vi "PicoScope5000aGetTriggerInfo.vi"(0 "handle in":i16, 5 "Rapid Block Acquisition Settings":T2 {"toSegmentIndex" format="%.4p"; "fromSegmentIndex" format="%.4p"}, 9 "Sample Rate":sgl, 11 "error in":errorcluster) -> (4 "handle out":i16, 6 "Trigger Info":T1(array[cluster]), 10 "Trigger Offsets":cluster{u64, sgl}[](array[cluster]) {"?" format="%#_5p"}, 15 "error out":errorcluster)   [LabVIEW 2010]
doc: "This VI gets a set of blocks captured using rapid block mode. It outputs two-dimensional arrays for each channel that contain data from all the requested captures."
uses:
  ps5000a.dll
  shared/Segment Range.ctl
panel:
  out "Number of Captures":u32=1
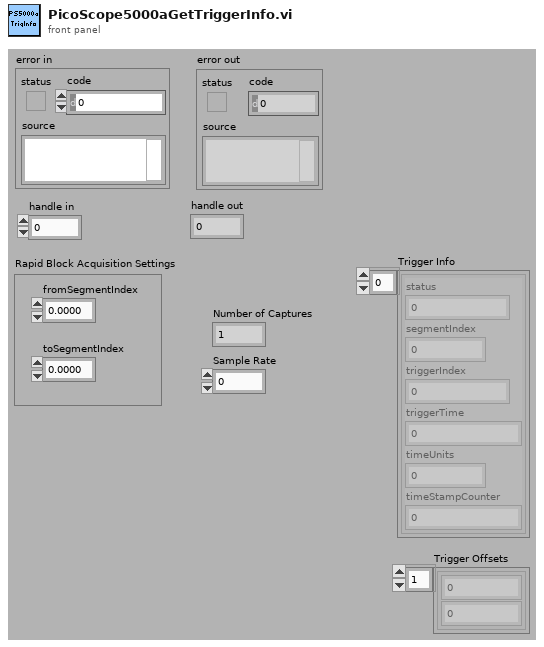
[diagram p1: front panel]
types:
  T1 = cluster{"status":u32, "segmentIndex":u32, "triggerIndex":u32, "triggerTime":i64, "timeUnits":i16, "timeStampCounter":u64}[]
  T2 = typedef "Segment Range.ctl" = cluster{"fromSegmentIndex":u64, "toSegmentIndex":u64}
  T3 = cluster{"status":u32, "segmentIndex":u32, "triggerIndex":u32, "triggerTime":i64, "timeUnits":i16, "reserved0":i16, "timeStampCounter":u64}
  T4 = cluster{"status":u32, "segmentIndex":u32, "triggerIndex":u32, "triggerTime":i64, "timeUnits":i16, "timeStampCounter":u64}
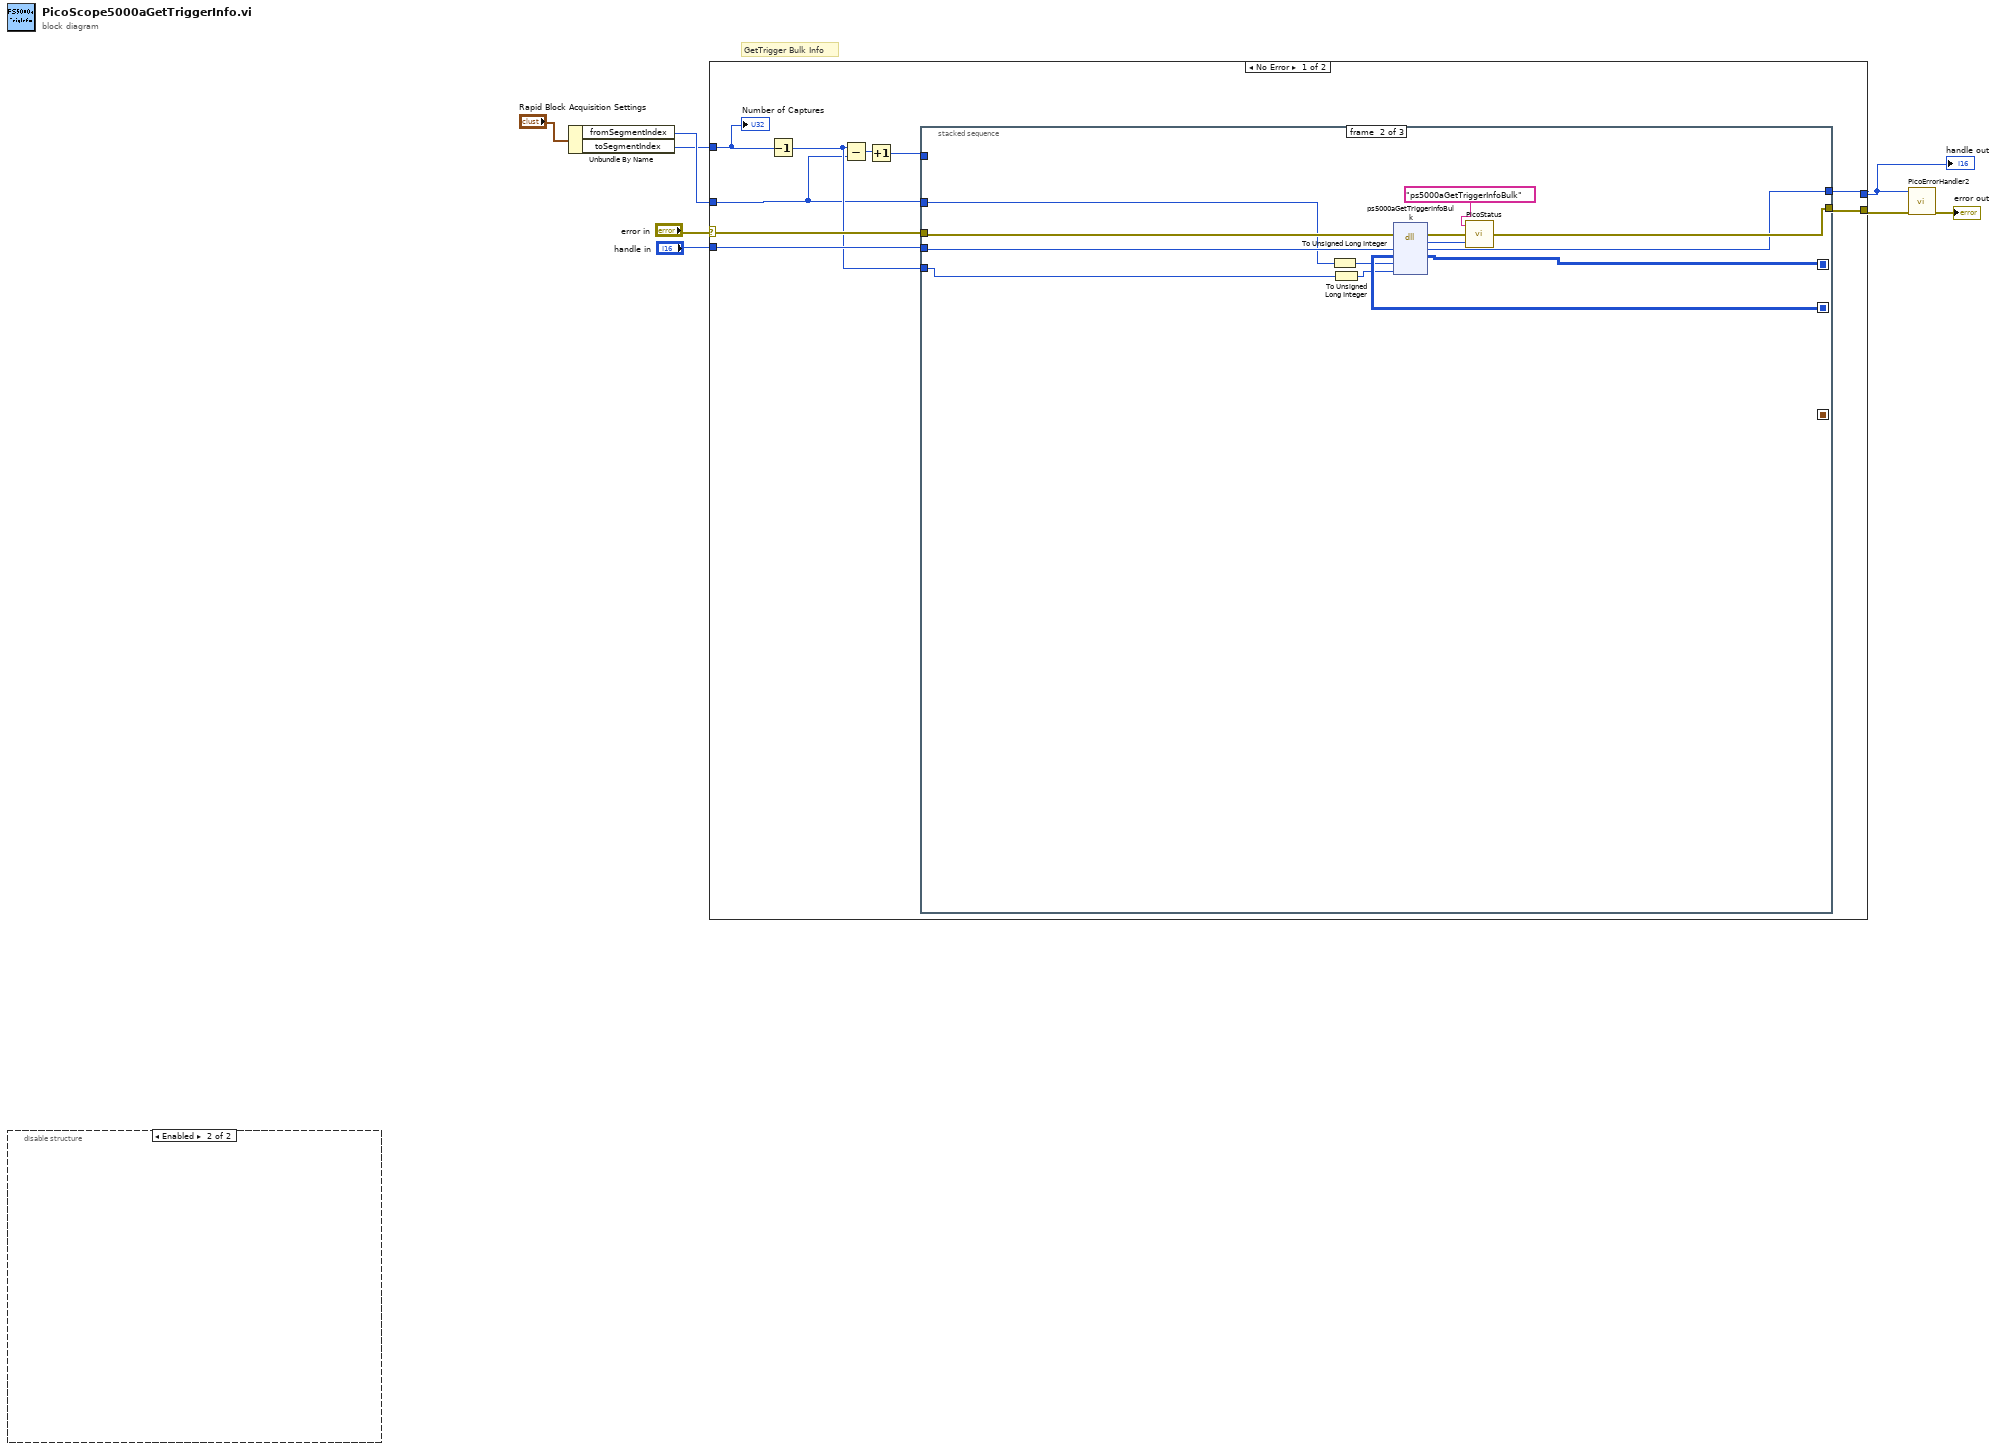
[diagram p0: block diagram]
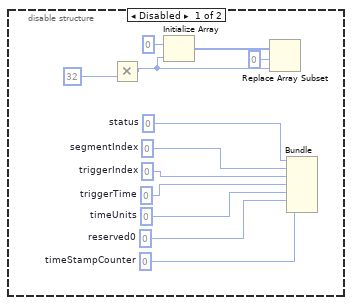
[diagram p2: hidden frame]
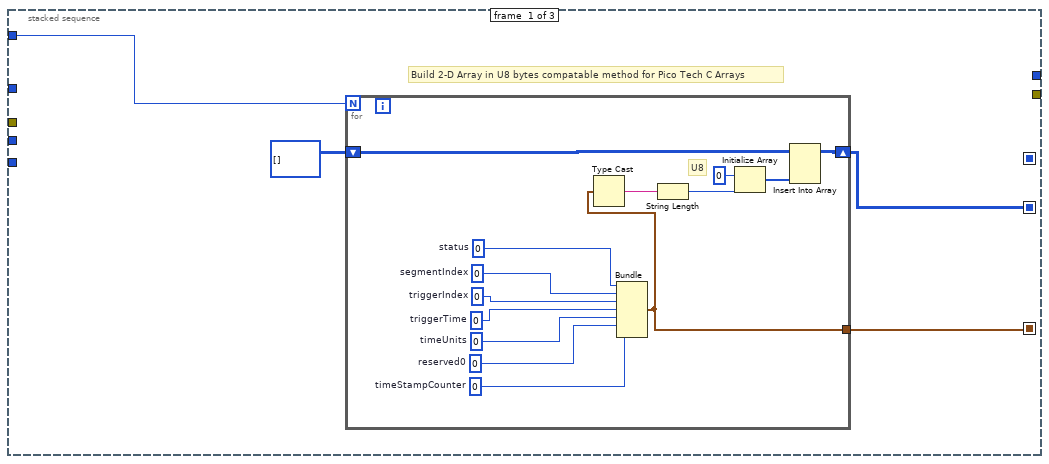
[diagram p3: hidden frame]
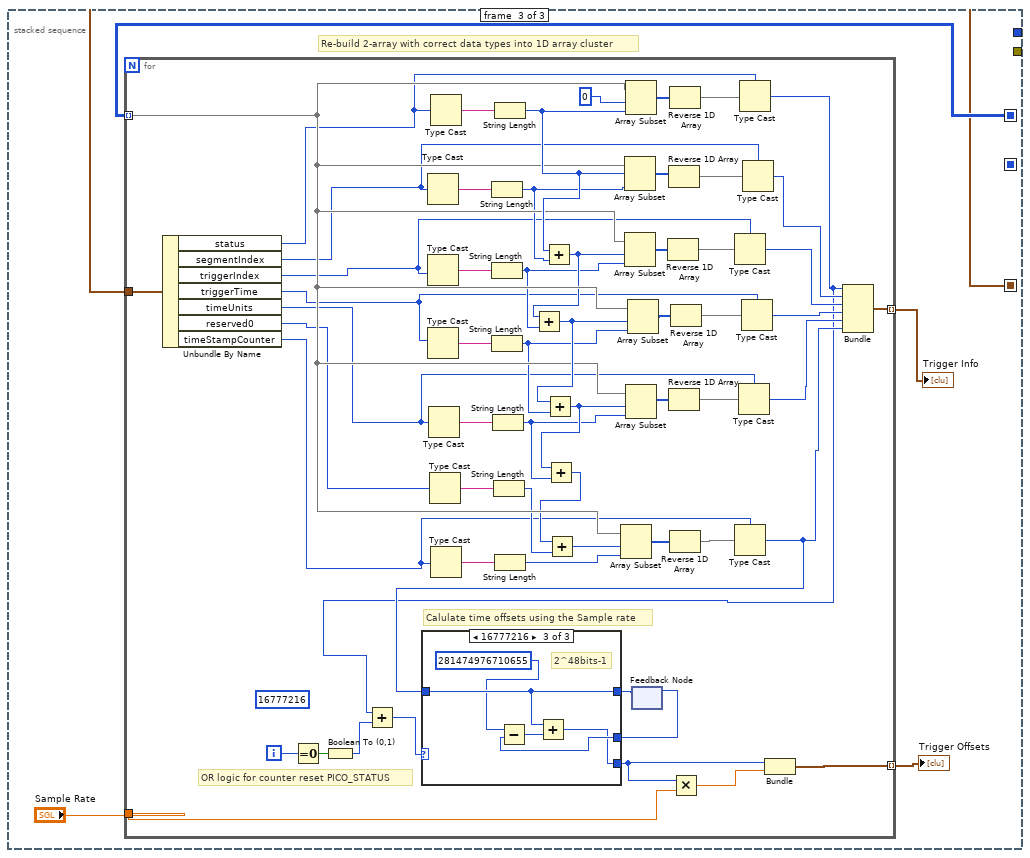
[diagram p4: hidden frame]
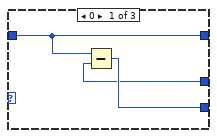
[diagram p5: hidden frame]
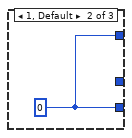
[diagram p6: hidden frame]
diagram:
  # "GetTrigger Bulk Info"
  n1 = disable-structure shown="Enabled" {
    frame Disabled {
      w16 = u64 0  # timeStampCounter
      w14 = i16 0  # reserved0
      w15 = i16 0  # timeUnits
      w17 = i64 0  # triggerTime
      w18 = u32 0  # triggerIndex
      w19 = u32 0  # segmentIndex
      w20 = u32 0  # status
      n2 = Multiply(y=u32 32) -> (x*y=w12:u32)  [unwired: 1 in]
      n3 = Initialize Array(u8 0 ("element"), w12) -> (w13:u8[])
      n4 = Replace Array Subset(array=w13, new element=w12, index=0) -> ()  [unwired: 1 out]
      n5 = Bundle("status"=w20, "segmentIndex"=w19, "triggerIndex"=w18, "triggerTime"=w17, "timeUnits"=w15, "reserved0"=w14, "timeStampCounter"=w16) -> ()  [unwired: 1 in, 1 out]
    }
    frame Enabled {
    }
  }
  n6 = Unbundle By Name("Rapid Block Acquisition Settings") -> ("fromSegmentIndex"=w2:u64, "toSegmentIndex"=w1:u64)
  n7 = case shown="No Error" "error in" {
    selector: "error in" -> [w28 w135]
    tunnel: [w25 w135] -> w5
    tunnel: "handle in" -> [w27 w134]
    tunnel: [w24 w134] -> w6
    tunnel: w1 -> [w29 _]
    tunnel: w2 -> [w21 _]
    frame No Error {
      n8 = Decrement(x=w29) -> (x-1=w26:u64)
      n9 = Subtract(x=w26, y=w21) -> (x-y=w23:u64)
      n10 = Increment(x=w23) -> (x+1=w22:u64)
      n11 = stacked-sequence {
        seq-local: [w31 _ _] -> [_ w55 _]
        seq-local: [w30 _ _] -> [_ w53 _]
        seq-local: [_ w54 _] -> [_ _ w66]
        seq-local: [_ w53 _] -> [_ _ w62]
        tunnel: w22 -> [w33 _ _]
        tunnel: w28 -> [_ w58 _]
        tunnel: w27 -> [_ w56 _]
        tunnel: w21 -> [_ w51 _]
        tunnel: w26 -> [_ w48 _]
        tunnel: [_ w57 _] -> w25
        tunnel: [_ w52 _] -> w24
        frame #0 {
          # "Build 2-D Array in U8 bytes compatable method for Pico Tech C Arrays"
          n12 = for {
            N: w33 -> [_]
            shift-right: [w35] -> w31
            shift-left: u8[][] [] -> [w36]
            tunnel: [w34] -> w30
            w43 = u64 0  # timeStampCounter
            w41 = i16 0  # reserved0
            w42 = i16 0  # timeUnits
            w44 = i64 0  # triggerTime
            w45 = u32 0  # triggerIndex
            w46 = u32 0  # segmentIndex
            w47 = u32 0  # status
            # "U8"
            n13 = Bundle("status"=w47, "segmentIndex"=w46, "triggerIndex"=w45, "triggerTime"=w44, "timeUnits"=w42, "reserved0"=w41, "timeStampCounter"=w43) -> (w34:T3)  [unwired: 1 in]
            n14 = Type Cast(x=w34) -> (*(type *) &x=w40:string)  [unwired: 1 in]
            n15 = String Length(string=w40) -> (length=w38:i32)
            n16 = Initialize Array(u8 0 ("element"), w38) -> (w37:u8[])
            n17 = Insert Into Array(array=w36, new element=w37) -> (w35:u8[][])  [unwired: 2 in]
          }
        }
        frame #1 {
          n18 = To Unsigned Long Integer(number=w51) -> (unsigned 32bit integer=w50:u32)
          n19 = To Unsigned Long Integer(number=w48) -> (unsigned 32bit integer=w49:u32)
          n20 = dll-call lib="ps5000a.dll" fn="ps5000aGetTriggerInfoBulk" ("ps3000.dll:_ps3000_open_unit@0")(error in=w58, "handle"=w56, "triggerInfo"=w55, "fromSegmentIndex"=w50, "toSegmentIndex"=w49) -> (error out=w61:errorcluster, "PICO_STATUS"=w60:u32, "handle"=w52:i16, "triggerInfo"=w54:u8[][])  [unwired: 4 in, 1 out]
          n21 = call "PicoStatus.vi"("PICO STATUS"=w60, "error in"=w61, "source"="ps5000aGetTriggerInfoBulk") -> ("error out"=w57:errorcluster)
        }
        frame #2 {
          # "Re-build 2-array with correct data types into 1D array cluster"
          n22 = for {
            tunnel: w66 -> [w86] mode=indexing
            tunnel: [w121] -> w65 mode=indexing
            tunnel: [w104] -> w64 mode=indexing
            tunnel: "Sample Rate" -> [w103]
            tunnel: w62 -> [w78]
            i -> [w107]
            (unwired) u32 16777216 ("status")
            # "Calulate time offsets using the Sample rate"
            # "OR logic for counter reset PICO_STATUS"
            n23 = Unbundle By Name(w78) -> ("status"=w77:u32, "segmentIndex"=w76:u32, "triggerIndex"=w71:u32, "triggerTime"=w72:i64, "timeUnits"=w73:i16, "reserved0"=w74:i16, "timeStampCounter"=w75:u64)
            n24 = Equal To 0?(x=w107) -> (x = 0?=w70:bool)
            n25 = Boolean To (0,1)(Boolean=w70) -> (0, 1=w69:i16)
            n26 = Type Cast(x=w76) -> (*(type *) &x=w99:string)  [unwired: 1 in]
            n27 = Type Cast(x=w71) -> (*(type *) &x=w98:string)  [unwired: 1 in]
            n28 = Type Cast(x=w72) -> (*(type *) &x=w97:string)  [unwired: 1 in]
            n29 = Type Cast(x=w73) -> (*(type *) &x=w96:string)  [unwired: 1 in]
            n30 = Type Cast(x=w74) -> (*(type *) &x=w95:string)  [unwired: 1 in]
            n31 = Type Cast(x=w77) -> (*(type *) &x=w100:string)  [unwired: 1 in]
            n32 = Type Cast(x=w75) -> (*(type *) &x=w90:string)  [unwired: 1 in]
            n33 = String Length(string=w99) -> (length=w84:i32)
            n34 = String Length(string=w98) -> (length=w82:i32)
            n35 = String Length(string=w97) -> (length=w81:i32)
            n36 = String Length(string=w96) -> (length=w80:i32)
            n37 = String Length(string=w95) -> (length=w79:i32)
            n38 = String Length(string=w100) -> (length=w91:i32)
            n39 = String Length(string=w90) -> (length=w88:i32)
            n40 = Add(x=w91, y=w84) -> (x+y=w83:i32)
            n41 = Add(x=w83, y=w82) -> (x+y=w94:i32)
            n42 = Add(x=w94, y=w81) -> (x+y=w93:i32)
            n43 = Add(x=w93, y=w80) -> (x+y=w85:i32)
            n44 = Add(x=w85, y=w79) -> (x+y=w89:i32)
            n45 = Array Subset(array=w86, index=w89, length=w88) -> (w87:u8[])
            n46 = Array Subset(array=w86, index=w91, length=w84) -> (w120:u8[])
            n47 = Array Subset(array=w86, index=w83, length=w82) -> (w115:u8[])
            n48 = Array Subset(array=w86, index=0, length=w91) -> (w118:u8[])
            n49 = Array Subset(array=w86, index=w93, length=w80) -> (w112:u8[])
            n50 = Array Subset(array=w86, index=w94, length=w81) -> (w114:u8[])
            n51 = feedback #1() -> (w105:u64)  [unwired: 1 in]
            n52 = Reverse 1D Array(array=w115) -> (reversed array=w116:u8[])
            n53 = Reverse 1D Array(array=w120) -> (reversed array=w119:u8[])
            n54 = Reverse 1D Array(array=w112) -> (reversed array=w111:u8[])
            n55 = Reverse 1D Array(array=w118) -> (reversed array=w117:u8[])
            n56 = Reverse 1D Array(array=w87) -> (reversed array=w110:u8[])
            n57 = Reverse 1D Array(array=w114) -> (reversed array=w113:u8[])
            n58 = Type Cast(type=w71, x=w116) -> (*(type *) &x=w124:u32)
            n59 = Type Cast(type=w75, x=w110) -> (*(type *) &x=w108:u64)
            n60 = Type Cast(type=w73, x=w111) -> (*(type *) &x=w122:i16)
            n61 = Type Cast(type=w77, x=w117) -> (*(type *) &x=w68:u32)
            n62 = Add(x=w68, y=w69) -> (x+y=w67:u32)
            n63 = case shown="16777216" w67 {
              tunnel: w108 -> [w126 _ w131]
              tunnel: [w126 w128 w131] -> w106
              tunnel: w105 -> [w125 _ w133]
              tunnel: [w127 w128 w129] -> w102
              frame 0 {
                n64 = Subtract(x=w126, y=w125) -> (x-y=w127:u64)
              }
              frame 1, Default {
                w128 = u64 0
              }
              frame 16777216 {
                # "2^48bits-1"
                n65 = Subtract(x=u64 281474976710655, y=w133) -> (x-y=w132:u64)
                n66 = Add(x=w131, y=w132) -> (x+y=w129:u64)
              }
            }
            n67 = feedback-in #1(w106) -> ()
            n68 = Multiply(x=w102, y=w103) -> (x*y=w101:sgl)
            n69 = Type Cast(type=w72, x=w113) -> (*(type *) &x=w123:i64)
            n70 = Type Cast(type=w76, x=w119) -> (*(type *) &x=w109:u32)
            n71 = Bundle(w102, w101) -> (w104:cluster{u64, sgl})  [unwired: 1 in]
            n72 = Bundle("status"=w68, "segmentIndex"=w109, "triggerIndex"=w124, "triggerTime"=w123, "timeUnits"=w122, "timeStampCounter"=w108) -> (w121:T4)  [unwired: 1 in]
          }
          "Trigger Info" <- w65
          "Trigger Offsets" <- w64
        }
      }
      "Number of Captures" <- w29
    }
    frame Error {
    }
  }
  "handle out" <- w6
  n73 = call "PicoErrorHandler2.vi"("error in (no error)"=w5, "handle In"=w6) -> ("error out"=→"error out":errorcluster)  [unwired: 9 in]
